vi "LoadProgram.vi"(0 "Universal Robot.lvclass in":refnum<class "Universal Robot.lvclass">, 1 "program in":string, 5 "error in (no error)":errorcluster, 8 "timeout (ms)":u32=5000) -> (14 "Universal Robot.lvclass out":refnum<class "Universal Robot.lvclass">, 15 "program out":string, 19 "error out":errorcluster)   [LabVIEW 2019, in "Universal Robot.lvclass"]
uses:
  Universal Robot.lvclass
  Universal Robot.lvclass/Universal Robot.ctl
  Client Interfaces/Dashboard Server/Dashboard Server.lvclass
panel:
  out "Load Time":u32
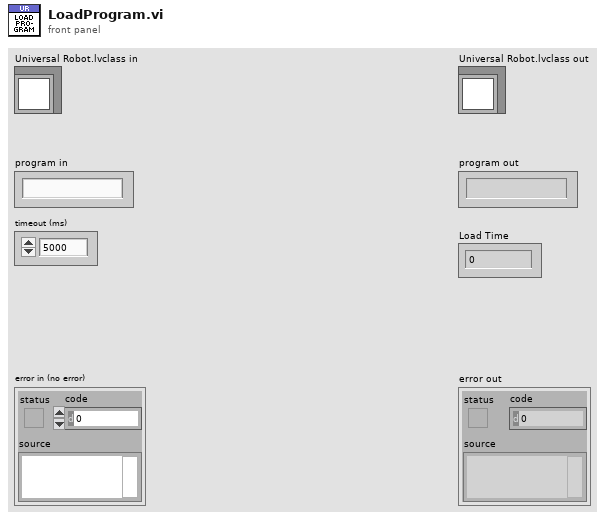
[diagram p1: front panel]
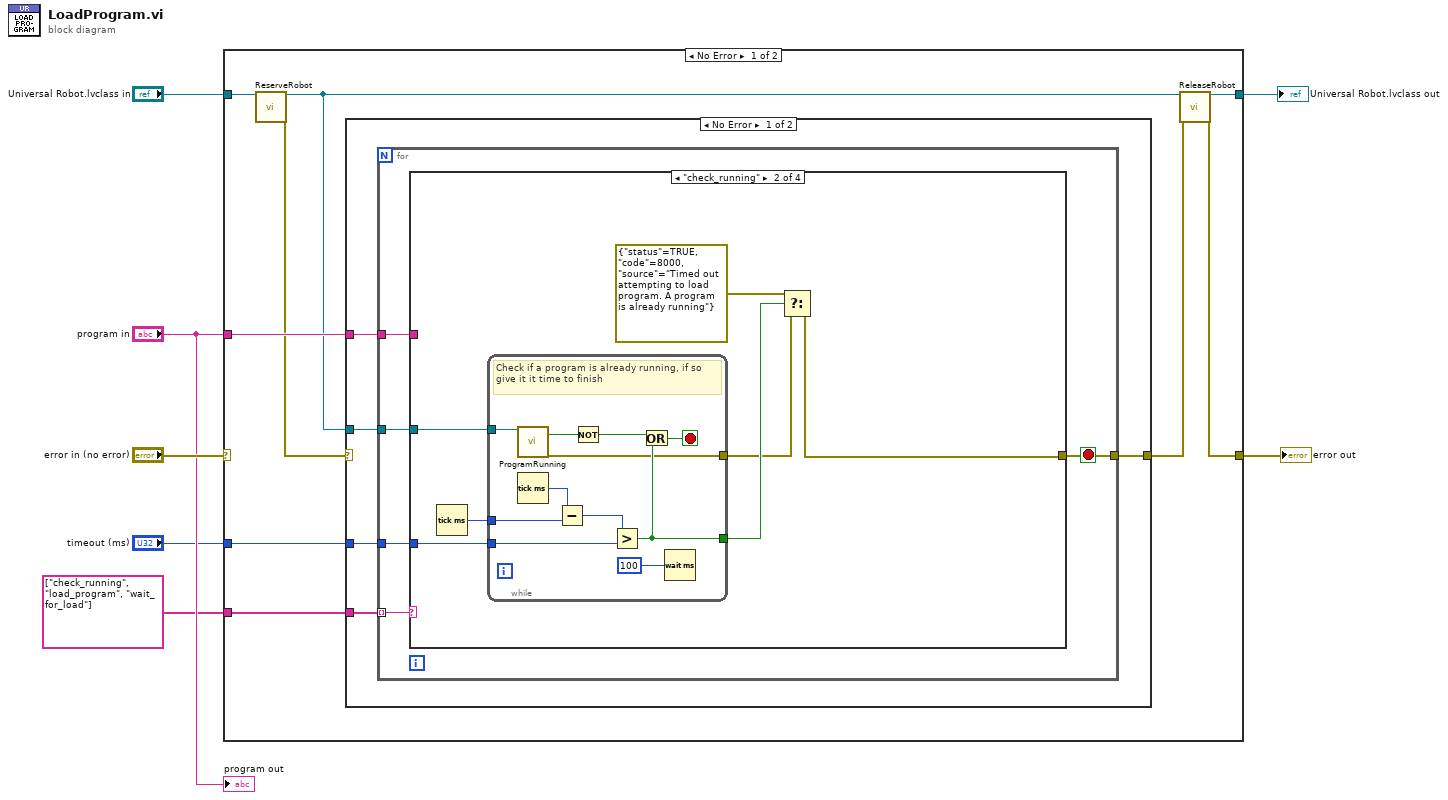
[diagram p0: block diagram]
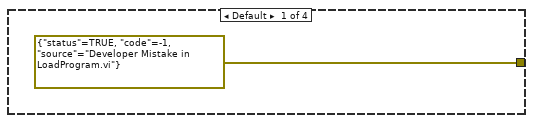
[diagram p2: hidden frame]
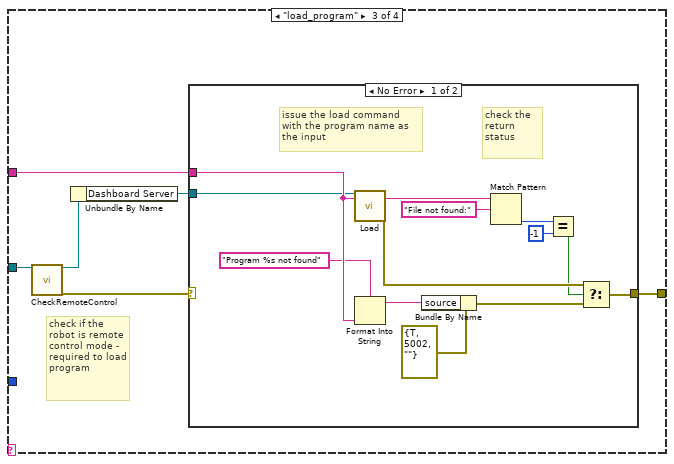
[diagram p3: hidden frame]
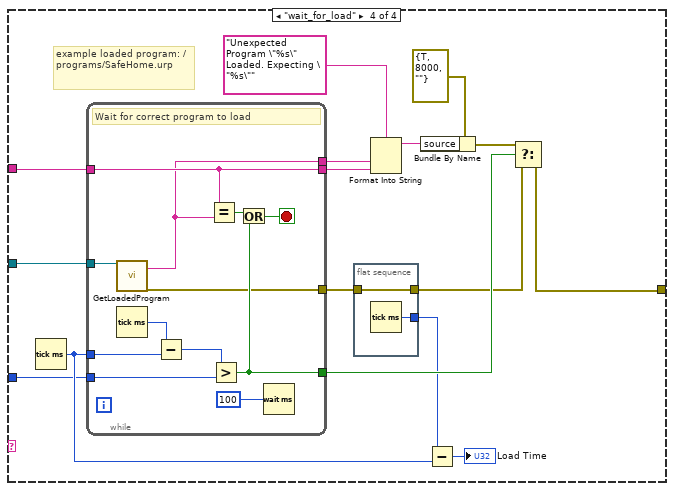
[diagram p5: hidden frame]
diagram:
  n1 = case shown="No Error" "error in (no error)" {
    selector: "error in (no error)" -> [_ w98]
    tunnel: [w8 w98] -> w5
    tunnel: "Universal Robot.lvclass in" -> [w13 w97]
    tunnel: [w10 w97] -> w4
    tunnel: "program in" -> [w16 _]
    tunnel: string[] ["check_running", "load_program", "wait_for_load"] -> [w15 _]
    tunnel: "timeout (ms)" -> [w14 _]
    frame No Error {
      n2 = call "ReserveRobot.vi"("Universal Robot.lvclass in"=w13) -> ("Universal Robot.lvclass out"=w11:refnum<class "Universal Robot.lvclass">, "error out"=w12:errorcluster)  [unwired: 17 in]
      n3 = case shown="No Error" w12 {
        selector: w12 -> [_ w96]
        tunnel: [w21 w96] -> w9
        tunnel: w16 -> [w20 _]
        tunnel: w15 -> [w19 _]
        tunnel: w14 -> [w18 _]
        tunnel: w11 -> [w17 _]
        frame No Error {
          n4 = for {
            tunnel: [w23] -> w21
            tunnel: w17 -> [w26]
            tunnel: w20 -> [w25]
            tunnel: w19 -> [w24] mode=indexing
            tunnel: w18 -> [w22]
            stop <- w23 stop-if-true
            n5 = case shown="\"check_running\"" w24 {
              tunnel: [errorcluster {"status"=TRUE, "code"=-1, "source"="Developer Mistake in LoadProgram.vi"} ("error out") w31 w51 w67] -> w23
              tunnel: w26 -> [_ w32 w50 w68]
              tunnel: w25 -> [_ _ w47 w81]
              tunnel: w22 -> [_ w30 _ w66]
              frame Default {
              }
              frame "check_running" {
                n6 = Tick Count (ms)() -> (millisecond timer value=w33:u32)
                n7 = while {
                  tunnel: w33 -> [w45]
                  tunnel: [w37] -> w28
                  tunnel: [w44] -> w34
                  tunnel: w32 -> [w38]
                  tunnel: w30 -> [w41]
                  stop <- w43 stop-if-true
                  # "Check if a program is already running, if so give it it time to finish"
                  n8 = call-dynamic "ProgramRunning.vi"("Universal Robot.lvclass in"=w38) -> ("running"=w36:bool, "error out"=w37:errorcluster)  [unwired: 16 in, 1 out]
                  n9 = Tick Count (ms)() -> (millisecond timer value=w40:u32)
                  n10 = Subtract(x=w40, y=w45) -> (x-y=w42:u32)
                  n11 = Not(x=w36) -> (.not. x?=w35:bool)
                  n12 = Greater?(x=w42, y=w41) -> (0:w44:bool)
                  n13 = Or(x=w35, y=w44) -> (x .or. y?=w43:bool)
                  n14 = Wait (ms)(milliseconds to wait=u32 100) -> ()  [unwired: 1 out]
                }
                n15 = Select(t=errorcluster {"status"=TRUE, "code"=8000, "source"="Timed out attempting to load program. A program is already running"} ("error constant"), s=w34, f=w28) -> (s? t:f=w31:errorcluster)
              }
              frame "load_program" {
                # "check if the robot is remote control mode - required to load program"
                n16 = call-dynamic "CheckRemoteControl.vi"("Universal Robot.lvclass in"=w50) -> ("Universal Robot.lvclass out"=w46:refnum<class "Universal Robot.lvclass">, "error out"=w48:errorcluster)  [unwired: 17 in]
                n17 = Unbundle By Name(w46) -> ("Dashboard Server"=w49:refnum<class "Dashboard Server.lvclass">)
                n18 = case shown="No Error" w48 {
                  selector: w48 -> [_ w65]
                  tunnel: [w64 w65] -> w51
                  tunnel: w49 -> [w62 _]
                  tunnel: w47 -> [w63 _]
                  frame No Error {
                    # "check the return status"
                    # "issue the load command with the program name as the input"
                    n19 = call-dynamic "Load.vi"("DashboardServer in"=w62, "program"=w63) -> ("returnStatus"=w61:string, "error out"=w57:errorcluster)  [unwired: 15 in, 1 out]
                    n20 = Format Into String(format string="Program %s not found", w63) -> (resulting string=w54:string)  [unwired: 2 in, 1 out]
                    n21 = Bundle By Name(cluster=errorcluster {"status"=TRUE, "code"=5002, "source"=""} ("error constant"), "source"=w54) -> (w53:errorcluster)
                    n22 = Match Pattern(string=w61, regular expression="File not found:") -> (offset past match=w59:i32)  [unwired: 1 in, 3 out]
                    n23 = Equal?(x=w59, y=-1) -> (x = y?=w56:bool)
                    n24 = Select(t=w57, s=w56, f=w53) -> (s? t:f=w64:errorcluster)
                  }
                  frame Error {
                  }
                }
              }
              frame "wait_for_load" {
                # "example loaded program: /programs/SafeHome.urp"
                n25 = Tick Count (ms)() -> (millisecond timer value=w71:u32)
                n26 = while {
                  tunnel: w71 -> [w95]
                  tunnel: [w85] -> w73
                  tunnel: [w94] -> w77
                  tunnel: w81 -> [w90]
                  tunnel: [w84] -> w80
                  tunnel: [w90] -> w79
                  tunnel: w68 -> [w86]
                  tunnel: w66 -> [w89]
                  stop <- w93 stop-if-true
                  # "Wait for correct program to load"
                  n27 = call-dynamic "GetLoadedProgram.vi"("Universal Robot.lvclass in"=w86) -> ("loaded program"=w84:string, "error out"=w85:errorcluster)  [unwired: 16 in, 1 out]
                  n28 = Tick Count (ms)() -> (millisecond timer value=w88:u32)
                  n29 = Subtract(x=w88, y=w95) -> (x-y=w92:u32)
                  n30 = Equal?(x=w90, y=w84) -> (x = y?=w91:bool)
                  n31 = Greater?(x=w92, y=w89) -> (0:w94:bool)
                  n32 = Or(x=w91, y=w94) -> (x .or. y?=w93:bool)
                  n33 = Wait (ms)(milliseconds to wait=u32 100) -> ()  [unwired: 1 out]
                }
                n34 = flat-sequence {
                  tunnel: w73 -> [w83]
                  tunnel: [w83] -> w72
                  tunnel: [w82] -> w70
                  frame #0 {
                    n35 = Tick Count (ms)() -> (millisecond timer value=w82:u32)
                  }
                }
                n36 = Format Into String(format string="Unexpected Program \"%s\" Loaded. Expecting \"%s\"", w80, w79) -> (resulting string=w75:string)  [unwired: 2 in, 1 out]
                n37 = Bundle By Name(cluster=errorcluster {"status"=TRUE, "code"=8000, "source"=""} ("error constant"), "source"=w75) -> (w74:errorcluster)
                n38 = Subtract(x=w70, y=w71) -> (x-y=→"Load Time":u32)
                n39 = Select(t=w74, s=w77, f=w72) -> (s? t:f=w67:errorcluster)
              }
            }
          }
        }
        frame Error {
        }
      }
      n40 = call "ReleaseRobot.vi"("Universal Robot.lvclass in"=w11, "error in (no error)"=w9) -> ("Universal Robot.lvclass out"=w10:refnum<class "Universal Robot.lvclass">, "error out"=w8:errorcluster)  [unwired: 16 in]
    }
    frame Error {
    }
  }
  "error out" <- w5
  "Universal Robot.lvclass out" <- w4
  "program out" <- "program in"
